vi "W32B Parse Spec.vi"(0 "function name":string, 5 "library path":path, 7 "parameters":string, 9 "links":string, 11 "error in":errorcluster) -> (4 "CLFN":T2, 6 "links out":T1(array[cluster]), 15 "error out":errorcluster)   [LabVIEW 2020]
doc: "Turns the text spec of one wrapper into the CLFN cluster and links array W32B Build Wrapper.vi takes. parameters: one line per CLFN parameter - the FIRST line is the return value - as name;Parameter Type;Numeric Type;Param Passing;Adapt Format[;Num Dimensions] with enum INDICES (Parameter Type 0 Numeric, 1 Array, 7 Any/adapt to type. Numeric Type 2 I32, 5 U16, 6 U32, 10 PTR INT, 11 PTR UINT. Param Passing 0 by value, 1 pointer to value. Adapt Format 0 handles by value. Num Dimensions is optional and only needed for an array parameter - 1 for a 1D array. A seventh field Array Passing is optional too: 0 Array Data Pointer (default), 1 Array Handle, 2 Array Handle Pointer). links: one line per wire as CLFN terminal;control label;node class;node source (1 output, 0 input)."
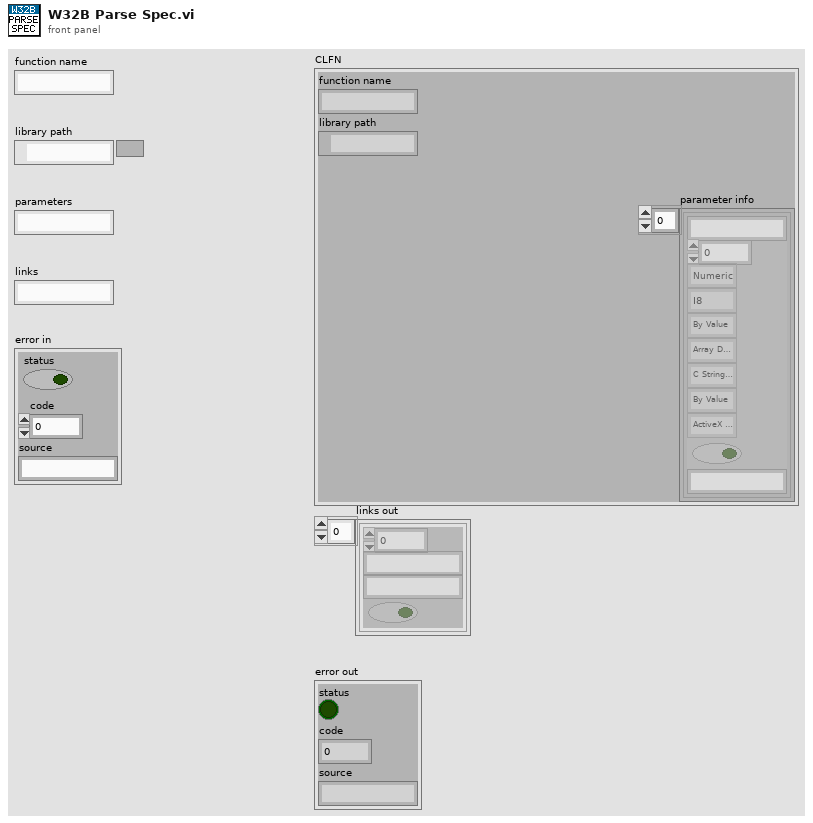
[diagram p1: front panel]
types:
  T1 = cluster{"CLFN terminal":i32, "control label":string, "node class":string, "node source?":bool}[]
  T2 = cluster{"function name":string, "library path":path, "parameter info":cluster{"Parameter Name":string, "Num Dimensions":i32, "Parameter Type":enum16{"Numeric", "Array", "String", "Waveform", "Digital Waveform", "Digital Table", "ActiveX", "Any", "Instance Data Pointer", "Void"}, "Numeric Type":enum16{"I8", "I16", "I32", "I64", "U8", "U16", "U32", "U64", "SGL", "DBL", "PTR INT", "PTR UINT"}, "Param Passing":enum16{"By Value", "Pointer To Value"}, "Array Passing":enum16{"Array Data Pointer", "Array Handle", "Array Handle Pointer"}, "String Passing":enum16{"C String Pointer", "Pascal String Pointer", "String Handle", "String Handle Pointer"}, "Adapt Format":enum16{"By Value", "Pointer To Value"}, "ActiveX Types":enum16{"ActiveX Variant Pointer", "IDispatch* Pointer", "IUnknown* Pointer"}, "Const (unused)":bool, "Minimum Size":string}[]}
  T3 = cluster{"CLFN terminal":i32, "control label":string, "node class":string, "node source?":bool}
  T4 = cluster{"Parameter Name":string, "Num Dimensions":i32, "Parameter Type":enum16{"Numeric", "Array", "String", "Waveform", "Digital Waveform", "Digital Table", "ActiveX", "Any", "Instance Data Pointer", "Void"}, "Numeric Type":enum16{"I8", "I16", "I32", "I64", "U8", "U16", "U32", "U64", "SGL", "DBL", "PTR INT", "PTR UINT"}, "Param Passing":enum16{"By Value", "Pointer To Value"}, "Array Passing":enum16{"Array Data Pointer", "Array Handle", "Array Handle Pointer"}, "String Passing":enum16{"C String Pointer", "Pascal String Pointer", "String Handle", "String Handle Pointer"}, "Adapt Format":enum16{"By Value", "Pointer To Value"}, "ActiveX Types":enum16{"ActiveX Variant Pointer", "IDispatch* Pointer", "IUnknown* Pointer"}, "Const (unused)":bool, "Minimum Size":string}
  T5 = cluster{"function name":string, "library path":path, cluster{"Parameter Name":string, "Num Dimensions":i32, "Parameter Type":enum16{"Numeric", "Array", "String", "Waveform", "Digital Waveform", "Digital Table", "ActiveX", "Any", "Instance Data Pointer", "Void"}, "Numeric Type":enum16{"I8", "I16", "I32", "I64", "U8", "U16", "U32", "U64", "SGL", "DBL", "PTR INT", "PTR UINT"}, "Param Passing":enum16{"By Value", "Pointer To Value"}, "Array Passing":enum16{"Array Data Pointer", "Array Handle", "Array Handle Pointer"}, "String Passing":enum16{"C String Pointer", "Pascal String Pointer", "String Handle", "String Handle Pointer"}, "Adapt Format":enum16{"By Value", "Pointer To Value"}, "ActiveX Types":enum16{"ActiveX Variant Pointer", "IDispatch* Pointer", "IUnknown* Pointer"}, "Const (unused)":bool, "Minimum Size":string}[]}
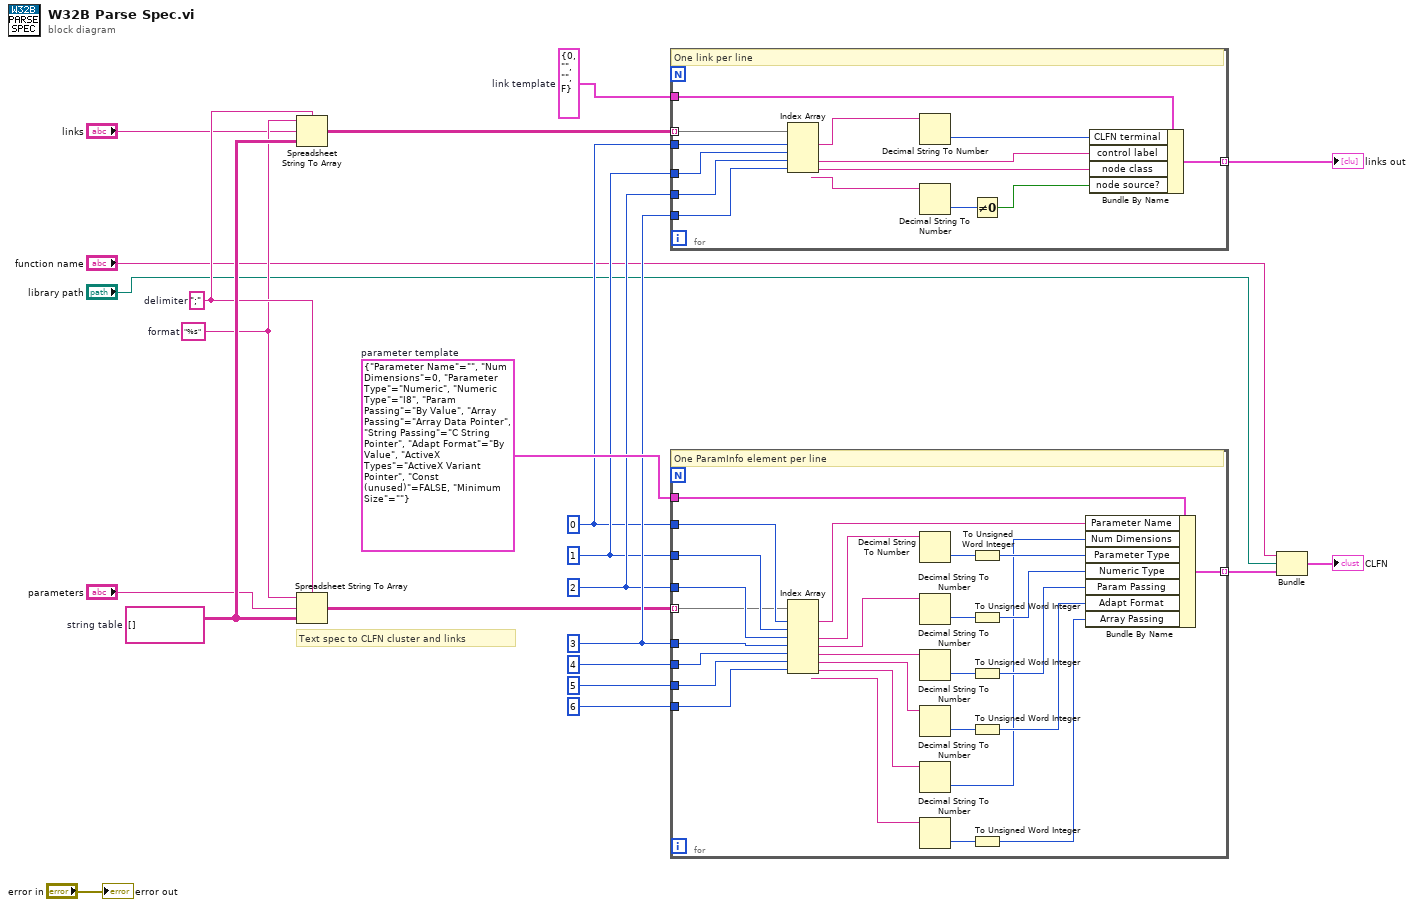
[diagram p0: block diagram]
diagram:
  w21 = T3 {"CLFN terminal"=0, "control label"="", "node class"="", "node source?"=FALSE}  # link template
  w20 = T4 {"Parameter Name"="", "Num Dimensions"=0, "Parameter Type"=enum."Numeric", "Numeric Type"=enum."I8", "Param Passing"=enum."By Value", "Array Passing"=enum."Array Data Pointer", "String Passing"=enum."C String Pointer", "Adapt Format"=enum."By Value", "ActiveX Types"=enum."ActiveX Variant Pointer", "Const (unused)"=FALSE, "Minimum Size"=""}  # parameter template
  w16 = 3
  w15 = 2
  w14 = 1
  w13 = 0
  w10 = string[][] []  # string table
  w9 = ";"  # delimiter
  w8 = "%s"  # format
  # "Text spec to CLFN cluster and links"
  n1 = Spreadsheet String To Array(delimiter (Tab)=w9, format string=w8, spreadsheet string="links", array type (2D Dbl)=w10) -> (array=w12:string[][])
  n2 = Spreadsheet String To Array(delimiter (Tab)=w9, format string=w8, spreadsheet string="parameters", array type (2D Dbl)=w10) -> (array=w11:string[][])
  n3 = for {
    tunnel: w21 -> [w24]
    tunnel: w13 -> [w25]
    tunnel: w14 -> [w26]
    tunnel: w15 -> [w27]
    tunnel: w16 -> [w28]
    tunnel: w12 -> [w23] mode=indexing
    tunnel: [w36] -> w7 mode=indexing
    # "One link per line"
    n4 = Index Array(array=w23, index #1=w25, index #2=w26, index #3=w27, index #4=w28) -> (element #1=w29:string, element #2=w30:string, element #3=w31:string, element #4=w32:string)
    n5 = Decimal String To Number(string=w29) -> (number=w33:i32)  [unwired: 2 in, 1 out]
    n6 = Decimal String To Number(string=w32) -> (number=w34:i32)  [unwired: 2 in, 1 out]
    n7 = Not Equal To 0?(x=w34) -> (x != 0?=w35:bool)
    n8 = Bundle By Name(cluster=w24, "CLFN terminal"=w33, "control label"=w30, "node class"=w31, "node source?"=w35) -> (w36:T3)
  }
  "links out" <- w7
  n9 = for {
    tunnel: w20 -> [w38]
    tunnel: w13 -> [w39]
    tunnel: w14 -> [w40]
    tunnel: w15 -> [w41]
    tunnel: w16 -> [w42]
    tunnel: 4 -> [w43]
    tunnel: 5 -> [w44]
    tunnel: 6 -> [w45]
    tunnel: w11 -> [w37] mode=indexing
    tunnel: [w64] -> w22 mode=indexing
    # "One ParamInfo element per line"
    n10 = Index Array(array=w37, index #1=w39, index #2=w40, index #3=w41, index #4=w42, index #5=w43, index #6=w44, index #7=w45) -> (element #1=w46:string, element #2=w47:string, element #3=w48:string, element #4=w49:string, element #5=w50:string, element #6=w51:string, element #7=w52:string)
    n11 = Decimal String To Number(string=w47) -> (number=w53:i32)  [unwired: 2 in, 1 out]
    n12 = Decimal String To Number(string=w48) -> (number=w54:i32)  [unwired: 2 in, 1 out]
    n13 = Decimal String To Number(string=w49) -> (number=w55:i32)  [unwired: 2 in, 1 out]
    n14 = Decimal String To Number(string=w50) -> (number=w56:i32)  [unwired: 2 in, 1 out]
    n15 = Decimal String To Number(string=w51) -> (number=w57:i32)  [unwired: 2 in, 1 out]
    n16 = Decimal String To Number(string=w52) -> (number=w58:i32)  [unwired: 2 in, 1 out]
    n17 = To Unsigned Word Integer(number=w53) -> (unsigned 16bit integer=w60:u16)
    n18 = To Unsigned Word Integer(number=w54) -> (unsigned 16bit integer=w61:u16)
    n19 = To Unsigned Word Integer(number=w55) -> (unsigned 16bit integer=w62:u16)
    n20 = To Unsigned Word Integer(number=w56) -> (unsigned 16bit integer=w63:u16)
    n21 = To Unsigned Word Integer(number=w58) -> (unsigned 16bit integer=w59:u16)
    n22 = Bundle By Name(cluster=w38, "Parameter Name"=w46, "Num Dimensions"=w57, "Parameter Type"=w60, "Numeric Type"=w61, "Param Passing"=w62, "Adapt Format"=w63, "Array Passing"=w59) -> (w64:T4)
  }
  n23 = Bundle("function name"="function name", "library path"="library path", w22) -> (→"CLFN":T5)  [unwired: 1 in]
  "error out" <- "error in"
